vi "VIH HelpGen - FILE - List Folder (with special exclusion & order spec).vi"(6 "pattern":string, 8 "error in":errorcluster, 10 "order file name":string, 11 "path":path) -> (0 "error out":errorcluster, 2 "File paths":path[](array[path]), 3 "path out":path)   [LabVIEW 2014]
doc: "::: VI Helpeks :::\nCopyright (c) 2000-2026 Konstantin Shifershteyn. All rights reserved."
panel:
  # "VI Helpeks\nCopyright (c) 2012-2026 Konstantin Shifershteyn"
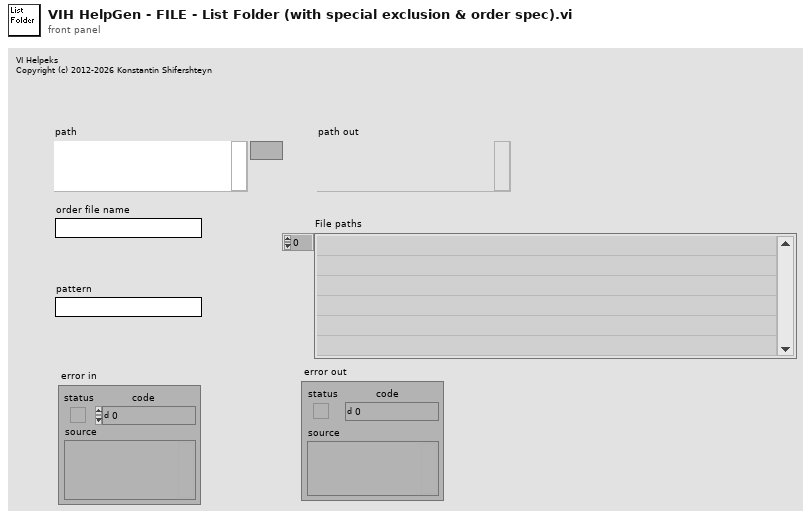
[diagram p1: front panel]
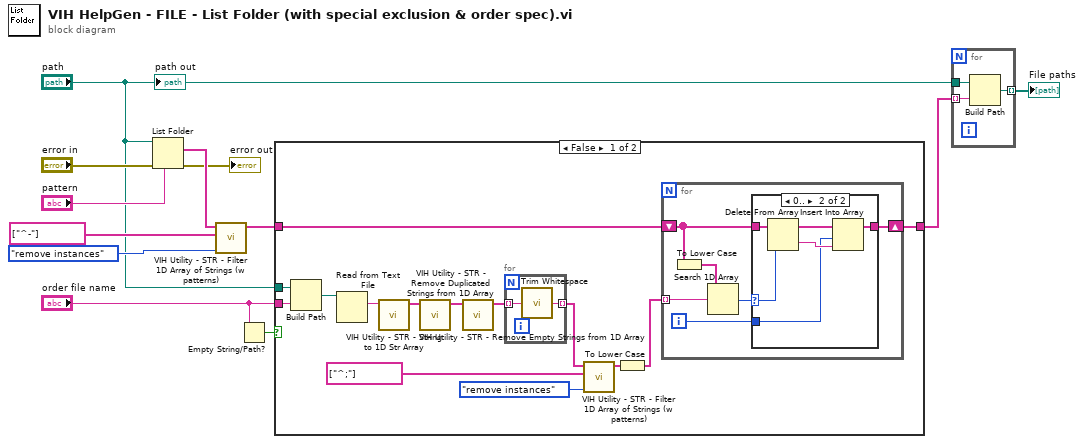
[diagram p0: block diagram]
diagram:
  n1 = List Folder(path="path", pattern="pattern", error in="error in") -> (filenames=w11:string[], error out=→"error out":errorcluster)  [unwired: 1 in, 2 out]
  n2 = call "VIH Utility - STR - Filter 1D Array of Strings (w patterns).vi"("Action (keep instances)"=enum16{"keep instances", "remove instances"}."remove instances", "Regular expressions"=string[] ["^-"], "Array in"=w11) -> ("Array out"=w1:string[])  [unwired: 8 in]
  n3 = Empty String/Path?(string/path="order file name") -> (empty?=w4:bool)
  n4 = case shown="False" w4 {
    tunnel: "path" -> [w26 _]
    tunnel: "order file name" -> [w25 _]
    tunnel: [w14 w42] -> w2
    tunnel: w1 -> [w13 w42]
    frame False {
      n5 = Build Path(base path=w26, name or relative path=w25) -> (appended path=w24:path)
      n6 = Read from Text File(file (use dialog)=w24) -> (text=w23:string)  [unwired: 3 in, 3 out]
      n7 = call "VIH Utility - STR - String to 1D Str Array.vi"("String in"=w23) -> ("Array out"=w22:string[])  [unwired: 6 in]
      n8 = call "VIH Utility - STR - Remove Empty Strings from 1D Array.vi"("String array in"=w22) -> ("String array out"=w21:string[])  [unwired: 9 in, 1 out]
      n9 = call "VIH Utility - STR - Remove Duplicated Strings from 1D Array.vi"("Array in"=w21) -> ("Array out"=w20:string[])  [unwired: 9 in, 1 out]
      n10 = for {
        tunnel: w20 -> [w41] mode=indexing
        tunnel: [w40] -> w17 mode=indexing
        n11 = call <vilib>:"Trim Whitespace.vi"("string"=w41) -> ("trimmed string"=w40:string)  [unwired: 1 in]
      }
      n12 = call "VIH Utility - STR - Filter 1D Array of Strings (w patterns).vi"("Action (keep instances)"=enum16{"keep instances", "remove instances"}."remove instances", "Regular expressions"=string[] ["^;"], "Array in"=w17) -> ("Array out"=w16:string[])  [unwired: 8 in]
      n13 = To Lower Case(string=w16) -> (all lower case string=w15:string[])
      n14 = for {
        shift-right: [w31] -> w14
        shift-left: w13 -> [w29]
        tunnel: w15 -> [w32] mode=indexing
        i -> [w30]
        n15 = To Lower Case(string=w29) -> (all lower case string=w28:string[])
        n16 = Search 1D Array(1D array=w28, element=w32) -> (index of element=w27:i32)  [unwired: 1 in]
        n17 = case shown="0.." w27 {
          selector: w27 -> [_ w34]
          tunnel: [w33 w38] -> w31
          tunnel: w30 -> [_ w36]
          tunnel: w29 -> [w33 w35]
          frame ..-1 {
          }
          frame 0.. {
            n18 = Delete From Array(array=w35, index=w34) -> (deleted portion=w37:string, array with subset deleted=w39:string[])  [unwired: 1 in]
            n19 = Insert Into Array(array=w39, index=w36, new element=w37) -> (w38:string[])
          }
        }
      }
    }
    frame True {
    }
  }
  n20 = for {
    tunnel: w2 -> [w45] mode=indexing
    tunnel: "path" -> [w44]
    tunnel: [w43] -> w6 mode=indexing
    n21 = Build Path(base path=w44, name or relative path=w45) -> (appended path=w43:path)
  }
  "File paths" <- w6
  "path out" <- "path"
